vi "Key_Send.vi"(0 "Channels":T1, 1 "History":i32, 5 "ScanCode":i32=-1, 7 "Released":bool, 9 "Quit":bool, 11 "error in":errorcluster) -> (4 "Quit out":bool, 6 "History out":i32, 15 "error out":errorcluster)   [LabVIEW 2020, in "GH_App.lvlib"]
doc: "Translates a key (ScanCode = physical key, independent of the keyboard layout) into a game key and puts it into the key queue. Pressed: arrows, Space = Jump, Enter/N = Start, Esc/P = Pause; released: arrows = ReleaseL/ReleaseR/ReleaseV. The Stop button sends Quit. Quit out: the game ends (Stop, or Esc on the title screen - read from the last game state). History = the last four pressed ScanCodes (8 bit each); Z U L U in a row sends the key Cheat."
uses:
  GH_App.lvlib
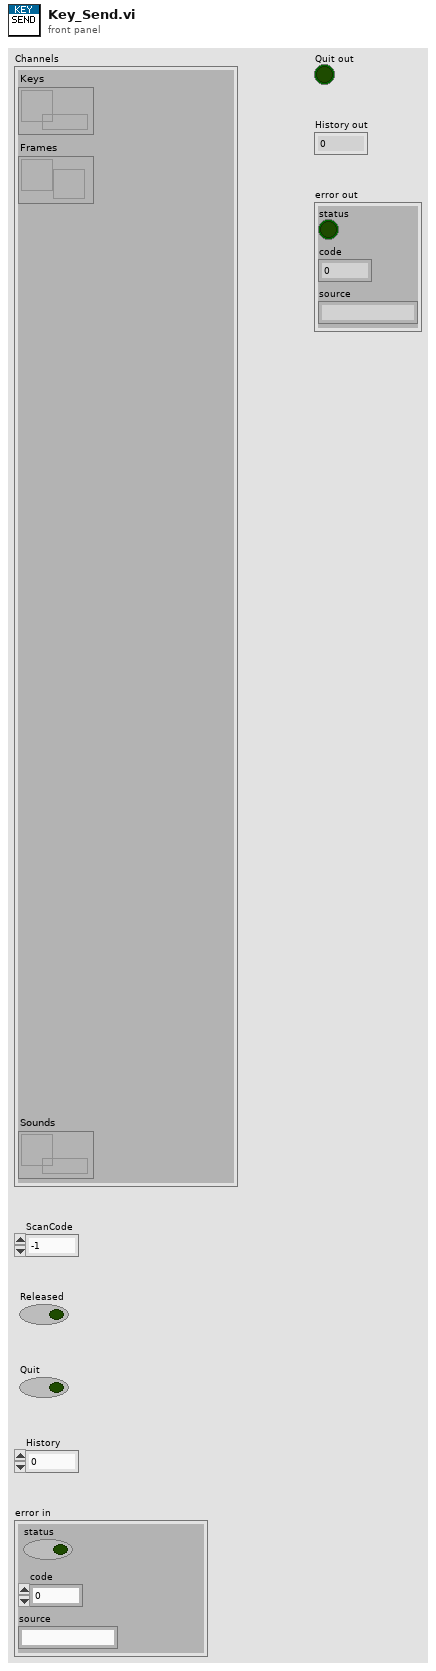
[diagram p1: front panel]
types:
  T1 = cluster{"Keys":refnum<queue>, "Frames":refnum<notifier>, "Sounds":refnum<queue>}
  T2 = cluster{"Tick":u32, "Phase":i32, "PhaseTicks":i32, "Level":i32, "Room":i32, "X10":i32, "Y10":i32, "VY10":i32, "Mode":i32, "Facing":i32, "Run":i32, "Vert":i32, "StandY":i32, "EntryX10":i32, "EntryY10":i32, "EntryMode":i32, "Lives":i32, "Score":i32, "NextLife":i32, "KeyR":i32, "KeyB":i32, "KeyY":i32, "Torch":bool, "FloorPhase":i32, "Dead":bool, "LevelStart":bool, "Quit":bool, "Sound":i32, "Seed":u32, "DemoStep":i32, "Tiles":u8[][], "World":cluster{"ID":string, "Depth":i32, "Column":i32, "Tiles":u8[][]}[], "Enemies":cluster{"Kind":i32, "X10":i32, "Y10":i32, "Dir":i32, "Mode":i32}[], "Highscores":cluster{"Score":i32, "Name":string}[], "Name":i32[], "Cursor":i32}
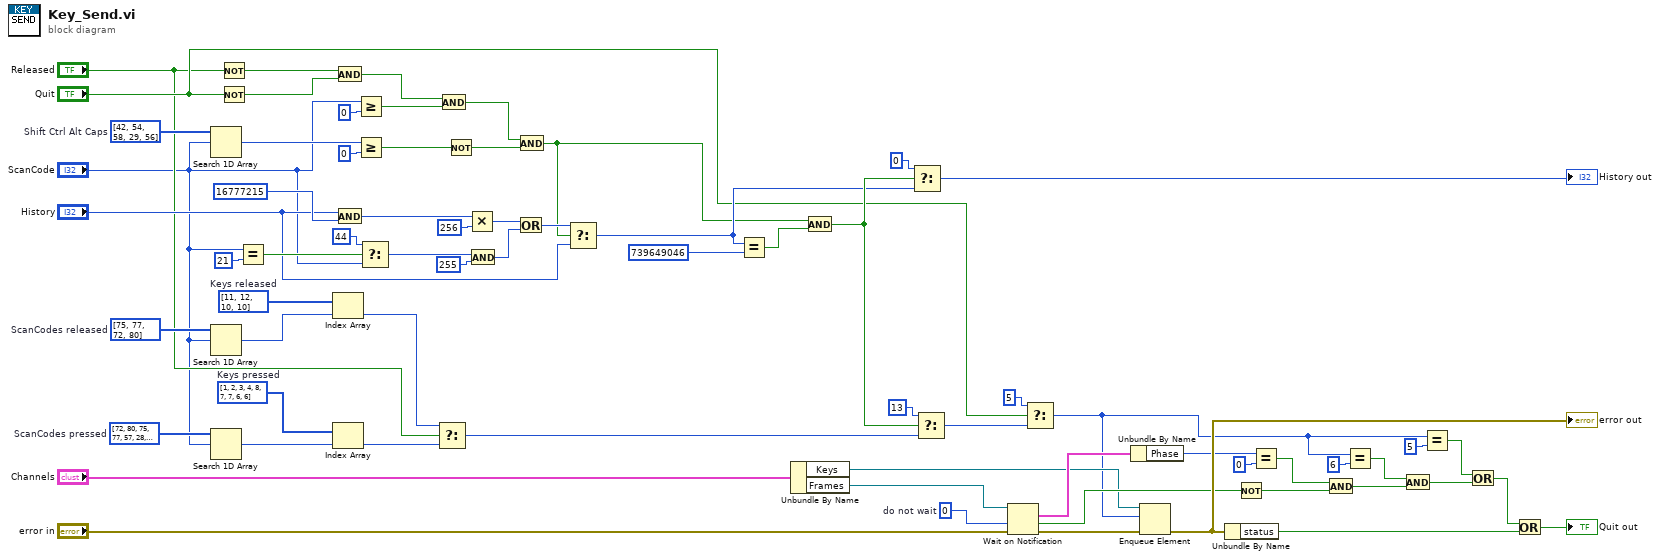
[diagram p0: block diagram]
diagram:
  w49 = 0  # do not wait
  w16 = i32[] [42, 54, 58, 29, 56]  # Shift Ctrl Alt Caps
  w12 = u16[] [1, 2, 3, 4, 8, 7, 7, 6, 6]  # Keys pressed
  w11 = i32[] [72, 80, 75, 77, 57, 28, 49, 1, 25]  # ScanCodes pressed
  w8 = u16[] [11, 12, 10, 10]  # Keys released
  w7 = i32[] [75, 77, 72, 80]  # ScanCodes released
  n1 = Search 1D Array(1D array=w16, element="ScanCode") -> (index of element=w17:i32)  [unwired: 1 in]
  n2 = Search 1D Array(1D array=w7, element="ScanCode") -> (index of element=w9:i32)  [unwired: 1 in]
  n3 = Search 1D Array(1D array=w11, element="ScanCode") -> (index of element=w13:i32)  [unwired: 1 in]
  n4 = Not(x="Released") -> (.not. x?=w20:bool)
  n5 = Not(x="Quit") -> (.not. x?=w21:bool)
  n6 = Equal?(x="ScanCode", y=21) -> (x = y?=w29:bool)
  n7 = Index Array(array=w8, index=w9) -> (element=w10:u16)
  n8 = Index Array(array=w12, index=w13) -> (element=w14:u16)
  n9 = And(x=w20, y=w21) -> (x .and. y?=w25:bool)
  n10 = And(x="History", y=16777215) -> (x .and. y?=w33:i32)
  n11 = Greater Or Equal?(x="ScanCode", y=0) -> (x >= y?=w23:bool)
  n12 = Greater Or Equal?(x=w17, y=0) -> (x >= y?=w19:bool)
  n13 = Select(t=44, s=w29, f="ScanCode") -> (s? t:f=w31:i32)
  n14 = Select(t=w10, s="Released", f=w14) -> (s? t:f=w15:u16)
  n15 = And(x=w25, y=w23) -> (x .and. y?=w26:bool)
  n16 = Not(x=w19) -> (.not. x?=w24:bool)
  n17 = Multiply(x=w33, y=256) -> (x*y=w35:i32)
  n18 = And(x=w31, y=255) -> (x .and. y?=w37:i32)
  n19 = Or(x=w35, y=w37) -> (x .or. y?=w38:i32)
  n20 = And(x=w26, y=w24) -> (x .and. y?=w27:bool)
  n21 = Select(t=w38, s=w27, f="History") -> (s? t:f=w39:i32)
  n22 = Equal?(x=w39, y=739649046) -> (x = y?=w41:bool)
  n23 = Unbundle By Name("Channels") -> ("Keys"=w47:refnum<queue>, "Frames"=w48:refnum<notifier>)
  n24 = And(x=w27, y=w41) -> (x .and. y?=w42:bool)
  n25 = Select(t=0, s=w42, f=w39) -> (s? t:f=→"History out":i32)
  n26 = Select(t=u16 13, s=w42, f=w15) -> (s? t:f=w44:u16)
  n27 = Wait on Notification(notifier=w48, timeout in ms (-1)=w49, error in (no error)="error in") -> (notification=w50:T2, timed out?=w51:bool, error out=w52:errorcluster)  [unwired: 1 in, 1 out]
  n28 = Select(t=u16 5, s="Quit", f=w44) -> (s? t:f=w46:u16)
  n29 = Unbundle By Name(w50) -> ("Phase"=w53:i32)
  n30 = Enqueue Element(queue=w47, element=w46, error in (no error)=w52) -> (error out=w54:errorcluster)  [unwired: 1 in, 2 out]
  "error out" <- w54
  n31 = Unbundle By Name(w54) -> ("status"=w65:bool)
  n32 = Not(x=w51) -> (.not. x?=w57:bool)
  n33 = Equal?(x=w53, y=0) -> (x = y?=w56:bool)
  n34 = And(x=w56, y=w57) -> (x .and. y?=w58:bool)
  n35 = Equal?(x=w46, y=u16 6) -> (x = y?=w62:bool)
  n36 = And(x=w62, y=w58) -> (x .and. y?=w63:bool)
  n37 = Equal?(x=w46, y=u16 5) -> (x = y?=w60:bool)
  n38 = Or(x=w60, y=w63) -> (x .or. y?=w64:bool)
  n39 = Or(x=w64, y=w65) -> (x .or. y?=→"Quit out":bool)
